vi "Moviment Preses.vi"(6 "y jugador":dbl, 9 "x jugador":dbl, 10 "y preses":dbl[](array[numeric]), 11 "x preses":dbl[](array[numeric])) -> (1 "Array":bool[](array[boolean]), 2 "y preses finals":dbl[](array[numeric]), 3 "x preses finals":dbl[](array[numeric]))   [LabVIEW 2023]
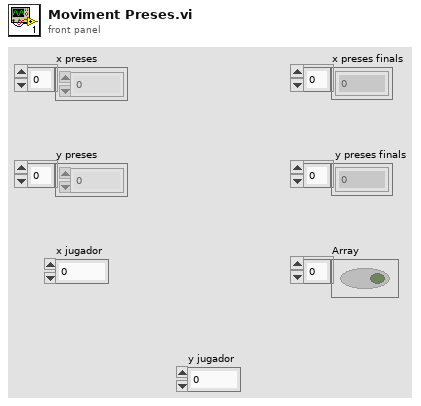
[diagram p1: front panel]
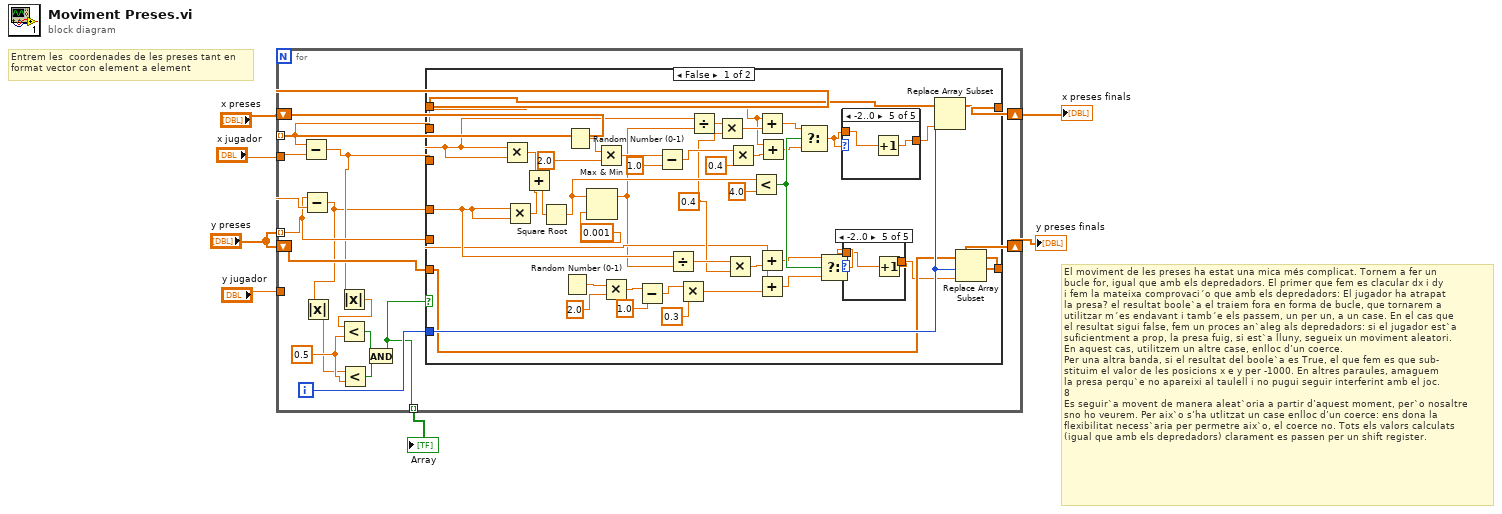
[diagram p0: block diagram]
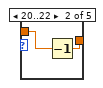
[diagram p3: hidden frame]
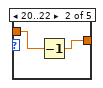
[diagram p7: hidden frame]
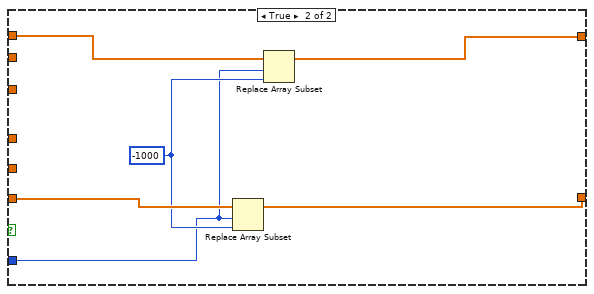
[diagram p10: hidden frame]
diagram:
  # "El moviment de les preses ha estat una mica més complicat. Tornem a fer un\nbucle for, igual que amb els depredadors. El primer que fem es clacular dx i dy\ni fem la mateixa comprovaci´o que amb els depredadors: El jugador ha atrapat\nla presa? el resultat boole`a el traiem fora en forma de bucle, que tornarem a\nutilitzar m´es endavant i tamb´e els passem, un per un, a un case. En el cas que\nel resultat sigui false, fem un proces an`aleg als depredadors: si el jugador est`a\nsuficientment a prop, la presa fuig, si est`a lluny, segueix un moviment aleatori.\nEn aquest cas, utilitzem un altre case, enlloc d’un coerce.\nPer una altra banda, si el resultat del boole`a es True, el que fem es que sub-\nstituim el valor de les posicions x e y per -1000. En altres paraules, amaguem\nla presa perqu`e no apareixi al taulell i no pugui seguir interferint amb el joc.\n8\nEs seguir`a movent de manera aleat`oria a partir d’aquest moment, per`o nosaltre\nsno ho veurem. Per aix`o s’ha utlitzat un case enlloc d’un coerce: ens dona la\nflexibilitat necess`aria per permetre aix`o, el coerce no. Tots els valors calculats\n(igual que amb els depredadors) clarament es passen per un shift register."
  # "Entrem les  coordenades de les preses tant en \nformat vector con element a element"
  n1 = for {
    tunnel: "x jugador" -> [w24]
    tunnel: "y jugador" -> [w19]
    tunnel: "x preses" -> [w18] mode=indexing
    tunnel: "y preses" -> [w14] mode=indexing
    shift-right: [w13] -> w5
    shift-left: "x preses" -> [w17]
    shift-right: [w15] -> w6
    shift-left: "y preses" -> [w16]
    tunnel: [w8] -> w7 mode=indexing
    i -> [w23]
    w22 = 0.5
    n2 = Subtract(x=w18, y=w24) -> (x-y=w11:dbl)
    n3 = Subtract(x=w14, y=w19) -> (x-y=w9:dbl)
    n4 = Absolute Value(x=w9) -> (abs(x)=w12:dbl)
    n5 = Absolute Value(x=w11) -> (abs(x)=w10:dbl)
    n6 = Less?(x=w10, y=w22) -> (x < y?=w21:bool)
    n7 = Less?(x=w12, y=w22) -> (x < y?=w20:bool)
    n8 = And(x=w21, y=w20) -> (x .and. y?=w8:bool)
    n9 = case shown="False" w8 {
      tunnel: w23 -> [w31 w83]
      tunnel: w18 -> [w36 _]
      tunnel: w14 -> [w38 _]
      tunnel: w11 -> [w37 _]
      tunnel: w9 -> [w39 _]
      tunnel: w17 -> [w35 w87]
      tunnel: w16 -> [w27 w88]
      tunnel: [w34 w86] -> w13
      tunnel: [w33 w85] -> w15
      frame False {
        w42 = 0.4
        n10 = Multiply(x=w37, y=w37) -> (x*y=w49:dbl)
        n11 = Multiply(x=w39, y=w39) -> (x*y=w50:dbl)
        n12 = Add(x=w49, y=w50) -> (x+y=w51:dbl)
        n13 = Square Root(x=w51) -> (sqrt(x)=w52:dbl)
        n14 = Random Number (0-1)() -> (number: 0 to 1=w57:dbl)
        n15 = Random Number (0-1)() -> (number: 0 to 1=w61:dbl)
        n16 = Max & Min(x=w52, y=0.001) -> (max(x,y)=w29:dbl)  [unwired: 1 out]
        n17 = Multiply(x=w61, y=2.0) -> (x*y=w62:dbl)
        n18 = Multiply(x=w57, y=2.0) -> (x*y=w58:dbl)
        n19 = Subtract(x=w58, y=1.0) -> (x-y=w59:dbl)
        n20 = Subtract(x=w62, y=1.0) -> (x-y=w63:dbl)
        n21 = Divide(x=w39, y=w29) -> (x/y=w53:dbl)
        n22 = Multiply(x=w59, y=0.3) -> (x*y=w60:dbl)
        n23 = Divide(x=w37, y=w29) -> (x/y=w54:dbl)
        n24 = Multiply(x=w54, y=w42) -> (x*y=w55:dbl)
        n25 = Multiply(x=w53, y=w42) -> (x*y=w56:dbl)
        n26 = Multiply(x=w63, y=0.4) -> (x*y=w64:dbl)
        n27 = Less?(x=w52, y=4.0) -> (x < y?=w68:bool)
        n28 = Add(x=w36, y=w55) -> (x+y=w32:dbl)
        n29 = Add(x=w38, y=w56) -> (x+y=w66:dbl)
        n30 = Add(x=w38, y=w60) -> (x+y=w65:dbl)
        n31 = Add(x=w36, y=w64) -> (x+y=w67:dbl)
        n32 = Select(t=w32, s=w68, f=w67) -> (s? t:f=w28:dbl)
        n33 = Select(t=w66, s=w68, f=w65) -> (s? t:f=w26:dbl)
        n34 = case shown="-2..0" w28 {
          tunnel: [w76 w77 w79 w80 w82] -> w30
          tunnel: w28 -> [w76 w78 w79 w80 w81]
          frame 1..19 {
          }
          frame 20..22 {
            n35 = Decrement(x=w78) -> (x-1=w77:dbl)
          }
          frame 23.. {
          }
          frame ..-3 {
          }
          frame -2..0 {
            n36 = Increment(x=w81) -> (x+1=w82:dbl)
          }
        }
        n37 = case shown="-2..0" w26 {
          tunnel: [w69 w70 w72 w73 w75] -> w25
          tunnel: w26 -> [w69 w71 w72 w73 w74]
          frame 1..19 {
          }
          frame 20..22 {
            n38 = Decrement(x=w71) -> (x-1=w70:dbl)
          }
          frame 23.. {
          }
          frame ..-3 {
          }
          frame -2..0 {
            n39 = Increment(x=w74) -> (x+1=w75:dbl)
          }
        }
        n40 = Replace Array Subset(array=w35, new element=w30, index=w31) -> (w34:dbl[])
        n41 = Replace Array Subset(array=w27, new element=w25, index=w31) -> (w33:dbl[])
      }
      frame True {
        w84 = -1000
        n42 = Replace Array Subset(array=w88, new element=w84, index=w83) -> (w85:dbl[])
        n43 = Replace Array Subset(array=w87, new element=w84, index=w83) -> (w86:dbl[])
      }
    }
  }
  "Array" <- w7
  "y preses finals" <- w6
  "x preses finals" <- w5
